vi "DUTModel.vi"(9 "Digital Input":bool, 10 "Power Supply Current":dbl format="%#_13g", 11 "Chamber Temp":dbl format="%#_13g") -> (1 "Digital Output":bool, 3 "Temps":T1)   [LabVIEW 2026]
uses:
  <vilib>/numeric/Random Number (Range) DBL.vi
  <vilib>/Analysis/baseanly.llb/Mean (DBL).vi
  <vilib>/Analysis/NI_AALBase.lvlib
  <vilib>/ptbypt/NI_PtbyPt.lvlib
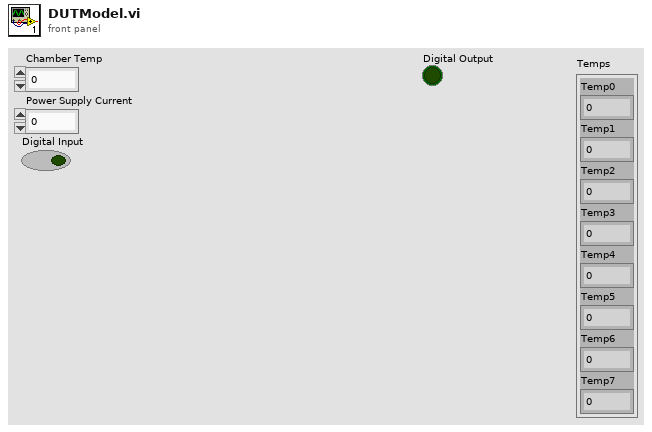
[diagram p1: front panel]
types:
  T1 = cluster{"Temp0":dbl, "Temp1":dbl, "Temp2":dbl, "Temp3":dbl, "Temp4":dbl, "Temp5":dbl, "Temp6":dbl, "Temp7":dbl}
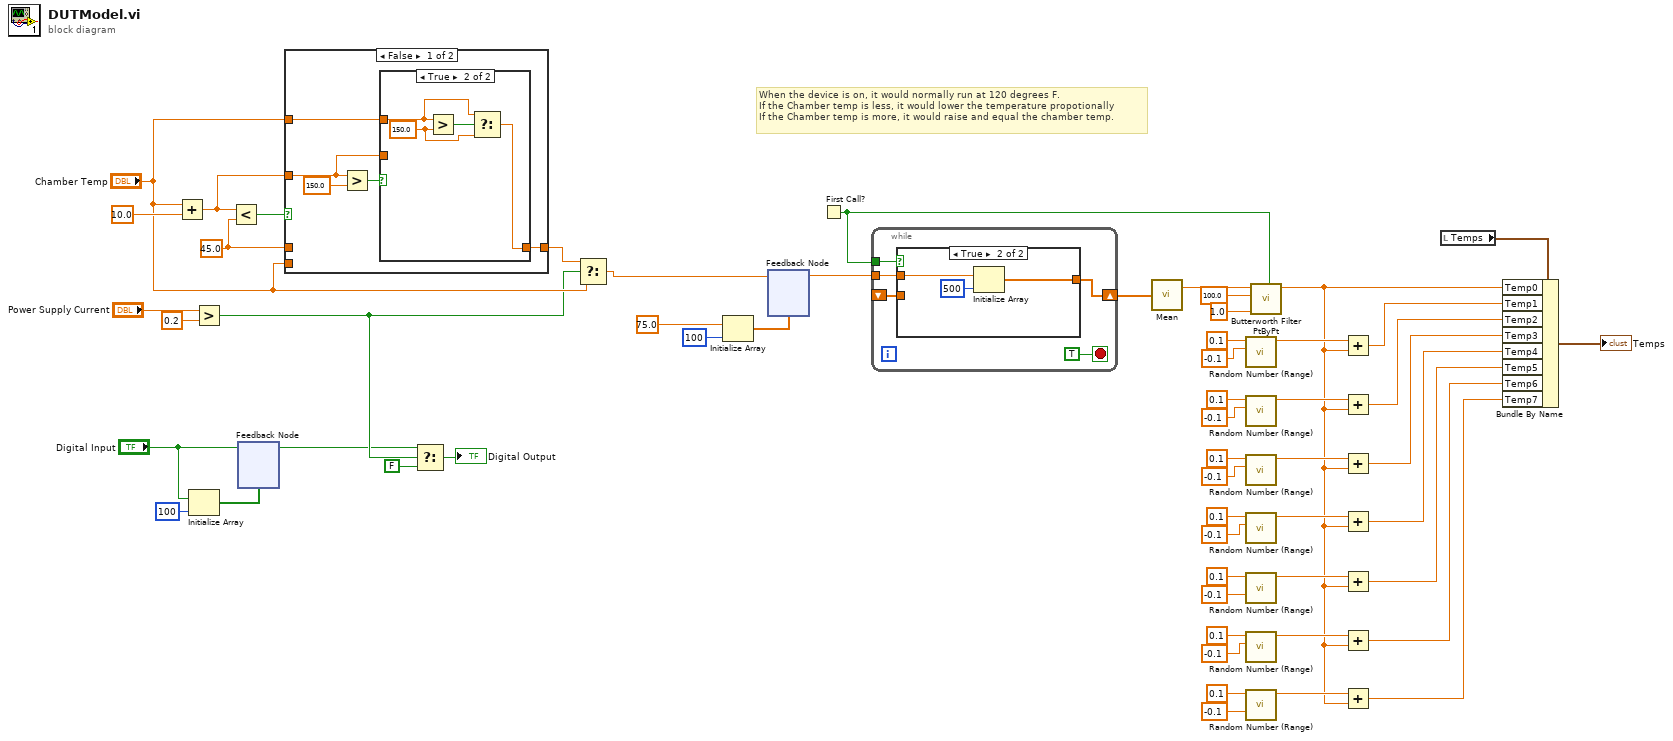
[diagram p0: block diagram]
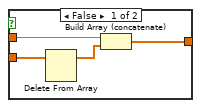
[diagram p2: hidden frame]
diagram:
  w44 = 45.0 ("lower limit")
  # "When the device is on, it would normally run at 120 degrees F.\nIf the Chamber temp is less, it would lower the temperature propotionally\nIf the Chamber temp is more, it would raise and equal the chamber temp."
  n1 = Add(x="Chamber Temp", y=10.0) -> (x+y=w42:dbl)
  n2 = Initialize Array("Digital Input", 100 ("dimension size")) -> (w54:bool[])
  n3 = Greater?(x="Power Supply Current", y=0.2) -> (0:w14:bool)
  n4 = Less?(x=w42, y=w44) -> (x < y?=w45:bool)
  n5 = feedback #1(w54) -> (w13:bool)
  n6 = feedback-in #1("Digital Input") -> ()
  n7 = case shown="False" w45 {
    tunnel: w44 -> [_ w67]
    tunnel: [w58 w67] -> w43
    tunnel: "Chamber Temp" -> [_ _]
    tunnel: w42 -> [w57 _]
    tunnel: "Chamber Temp" -> [w59 _]
    frame False {
      n8 = Greater?(x=w57, y=150.0) -> (0:w60:bool)
      n9 = case shown="True" w60 {
        tunnel: w59 -> [_ w65]
        tunnel: [w62 w64] -> w58
        tunnel: w57 -> [w62 _]
        frame False {
        }
        frame True {
          w63 = 150.0 ("y")
          n10 = Greater?(x=w65, y=w63) -> (0:w66:bool)
          n11 = Select(t=w65, s=w66, f=w63) -> (s? t:f=w64:dbl)
        }
      }
    }
    frame True {
    }
  }
  n12 = Select(t=w13, s=w14, f=FALSE) -> (s? t:f=→"Digital Output":bool)
  n13 = Select(t=w43, s=w14, f="Chamber Temp") -> (s? t:f=w40:dbl)
  n14 = Initialize Array(75.0 ("upper limit"), 100 ("dimension size")) -> (w49:dbl[])
  n15 = feedback #2(w49) -> (w38:dbl)
  n16 = feedback-in #2(w40) -> ()
  n17 = First Call?() -> (First Call?: T/F=w37:bool)
  n18 = while {
    tunnel: w38 -> [w72]
    tunnel: w37 -> [w71]
    shift-right: [w70] -> w36
    shift-left: _ -> [w69]
    stop <- TRUE stop-if-true
    n19 = case shown="True" w71 {
      tunnel: w72 -> [w75 w79]
      tunnel: [w73 w77] -> w70
      tunnel: w69 -> [w76 _]
      frame False {
        n20 = Delete From Array(array=w76) -> (array with subset deleted=w74:dbl[])  [unwired: 2 in, 1 out]
        n21 = Build Array (concatenate)(w75, w74) -> (w73:dbl[])
      }
      frame True {
        n22 = Initialize Array(w79, 500 ("dimension size")) -> (w77:dbl[])
      }
    }
  }
  n23 = call-poly <vilib>:"Mean.vi"("X"=w36) -> ("mean"=w48:dbl)  [unwired: 1 out]
  n24 = call-poly <vilib>:"Random Number (Range).vi"("lower bound (0)"=-0.1, "upper bound (100)"=0.1) -> ("number"=w22:dbl)  [unwired: 9 in]
  n25 = call-poly <vilib>:"Random Number (Range).vi"("lower bound (0)"=-0.1, "upper bound (100)"=0.1) -> ("number"=w21:dbl)  [unwired: 9 in]
  n26 = call-poly <vilib>:"Random Number (Range).vi"("lower bound (0)"=-0.1, "upper bound (100)"=0.1) -> ("number"=w20:dbl)  [unwired: 9 in]
  n27 = call-poly <vilib>:"Random Number (Range).vi"("lower bound (0)"=-0.1, "upper bound (100)"=0.1) -> ("number"=w19:dbl)  [unwired: 9 in]
  n28 = call-poly <vilib>:"Random Number (Range).vi"("lower bound (0)"=-0.1, "upper bound (100)"=0.1) -> ("number"=w18:dbl)  [unwired: 9 in]
  n29 = call-poly <vilib>:"Random Number (Range).vi"("lower bound (0)"=-0.1, "upper bound (100)"=0.1) -> ("number"=w17:dbl)  [unwired: 9 in]
  n30 = call-poly <vilib>:"Random Number (Range).vi"("lower bound (0)"=-0.1, "upper bound (100)"=0.1) -> ("number"=w16:dbl)  [unwired: 9 in]
  n31 = call <vilib>:"Butterworth Filter PtByPt.vi"("initialize"=w37, "low cutoff freq: fl"=1.0, "sampling freq: fs"=100.0, "x"=w48) -> ("Filtered x"=w8:dbl)  [unwired: 5 in, 1 out]
  n32 = Add(x=w22, y=w8) -> (x+y=w7:dbl)
  n33 = Add(x=w21, y=w8) -> (x+y=w6:dbl)
  n34 = Add(x=w20, y=w8) -> (x+y=w5:dbl)
  n35 = Add(x=w19, y=w8) -> (x+y=w4:dbl)
  n36 = Add(x=w18, y=w8) -> (x+y=w3:dbl)
  n37 = Add(x=w17, y=w8) -> (x+y=w2:dbl)
  n38 = Add(x=w16, y=w8) -> (x+y=w1:dbl)
  n39 = local read "Temps"() -> (w10:T1)
  n40 = Bundle By Name(cluster=w10, "Temp0"=w8, "Temp1"=w7, "Temp2"=w6, "Temp3"=w5, "Temp4"=w4, "Temp5"=w3, "Temp6"=w2, "Temp7"=w1) -> (→"Temps":T1)
